vi "AlarmText.vi"(11 "Code":u16) -> (3 "Text":string)   [LabVIEW 2018]
doc: "Use this template to build a VI to use as a subVI."
panel:
  # "說明：異常碼轉英文文字。"
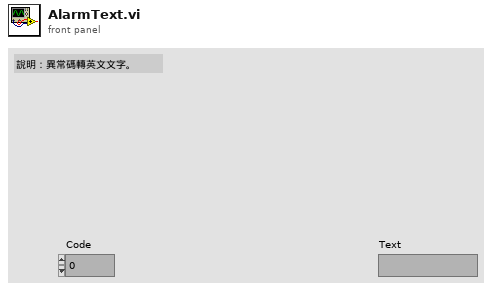
[diagram p1: front panel]
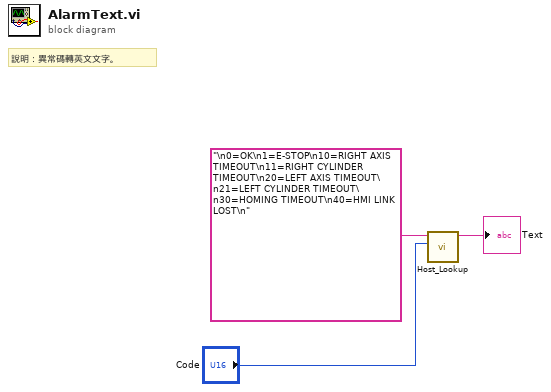
[diagram p0: block diagram]
diagram:
  # "說明：異常碼轉英文文字。"
  n1 = call "Host_Lookup.vi"("Key"="Code", "Table"="\n0=OK\n1=E-STOP\n10=RIGHT AXIS TIMEOUT\n11=RIGHT CYLINDER TIMEOUT\n20=LEFT AXIS TIMEOUT\n21=LEFT CYLINDER TIMEOUT\n30=HOMING TIMEOUT\n40=HMI LINK LOST\n") -> ("Text"=→"Text":string)  [unwired: 9 in]
